vi "Test_Sim_First_Order_Step_Caraya.vi"(8 "error in":errorcluster) -> (0 "error out":errorcluster)   [LabVIEW 2026]
doc: "Caraya test of Sim First Order Step.vi: 0->100 with dt 0.1 tau 0.8 gives 11.7503097415; an unchanged channel stays unchanged."
uses:
  <vilib>/addons/_JKI Toolkits/Caraya/classes/Test/Test.lvclass
  <vilib>/addons/_JKI Toolkits/Caraya/classes/Assert/Assert.lvclass
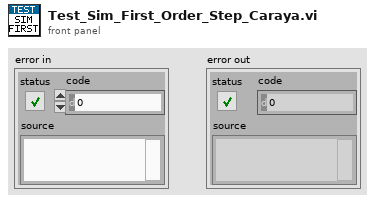
[diagram p1: front panel]
types:
  T1 = typedef "Channel Value.ctl" = cluster{"channel":string, "value":dbl}
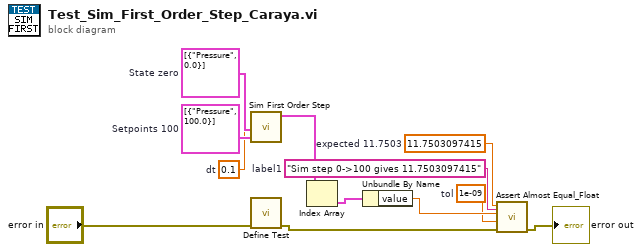
[diagram p0: block diagram]
diagram:
  w3 = "Sim step 0->100 gives 11.7503097415"  # label1
  w4 = 1e-09  # tol
  w6 = 11.7503097415  # expected 11.7503
  w9 = 0.1  # dt
  w10 = cluster{"channel":string, "value":dbl}[] [{"channel"="Pressure", "value"=100.0}]  # Setpoints 100
  w11 = cluster{"channel":string, "value":dbl}[] [{"channel"="Pressure", "value"=0.0}]  # State zero
  n1 = call "Sim First Order Step.vi"("dt s"=w9, "Setpoints"=w10, "State"=w11) -> ("new State"=w8:T1[])  [unwired: 8 in]
  n2 = call <vilib>:"Define Test.vi"("error in (no error)"="error in") -> ("error out"=w2:errorcluster)  [unwired: 9 in, 1 out]
  n3 = Index Array(array=w8) -> (element=w7:T1)  [unwired: 1 in]
  n4 = Unbundle By Name(w7) -> ("value"=w5:dbl)
  n5 = call <vilib>:"Assert Almost Equal_Float.vi"("Label"=w3, "error in (no error)"=w2, "Tolerance"=w4, "Actual"=w5, "Expected"=w6) -> ("error out"=→"error out":errorcluster)  [unwired: 5 in, 1 out]
